vi "NanonisScanAction.vi"(8 "error in (no error)":errorcluster, 11 "String input":string="string test") -> (0 "error out":errorcluster, 3 "String output":string)   [LabVIEW 2011]
uses:
  <userlib>/Nanonis Prog Interface/Nanonis Prog Interface.lvlib
panel:
  out "Application ref out":refnum<vi>
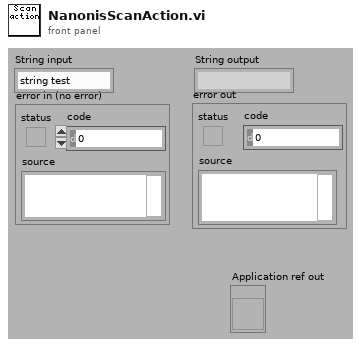
[diagram p1: front panel]
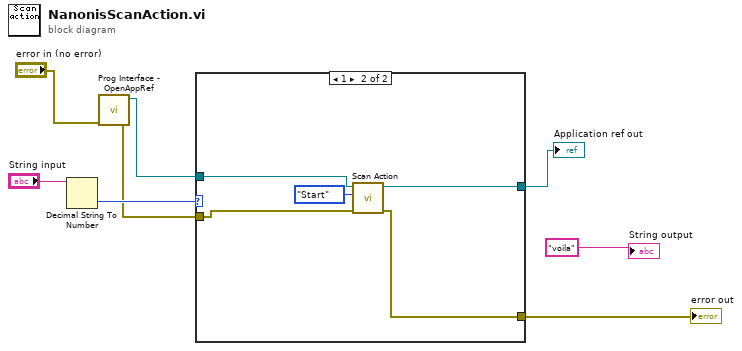
[diagram p0: block diagram]
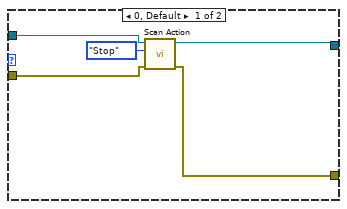
[diagram p2: hidden frame]
diagram:
  n1 = Decimal String To Number(string="String input") -> (number=w7:i32)  [unwired: 2 in, 1 out]
  n2 = call <userlib>:"Prog Interface - OpenAppRef.vi"("Error in (no error)"="error in (no error)") -> ("Error out"=w3:errorcluster, "Application reference"=w4:refnum<vi>)  [unwired: 5 in]
  n3 = case shown="1" w7 {
    tunnel: w3 -> [w12 w17]
    tunnel: [w11 w18] -> w6
    tunnel: [w10 w15] -> w5
    tunnel: w4 -> [w9 w14]
    frame 0, Default {
      n4 = call "Scan Action.vi"("error in (no error)"=w12, "Scan action (Start)"=enum16{"Start", "Stop", "Pause", "Resume"}."Stop", "Application ref in"=w9) -> ("error out"=w11:errorcluster, "Application ref out"=w10:refnum<vi>)  [unwired: 6 in]
    }
    frame 1 {
      n5 = call "Scan Action.vi"("error in (no error)"=w17, "Scan action (Start)"=enum16{"Start", "Stop", "Pause", "Resume"}."Start", "Application ref in"=w14) -> ("error out"=w18:errorcluster, "Application ref out"=w15:refnum<vi>)  [unwired: 6 in]
    }
  }
  "error out" <- w6
  "Application ref out" <- w5
  "String output" <- "voila"
